vi "PrimaryProviderExample_CreateNewWizard_Invoke.vi"(10 "Cluster":T1, 11 "Wizard":T2) -> (3 "Canceled":bool)   [LabVIEW 2023]
uses:
  <resource>/Framework/Providers/API/ItemRef.ctl
  <resource>/Framework/Providers/API/mxLvNIIM.ctl
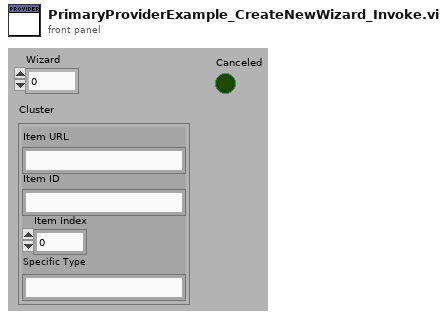
[diagram p1: front panel]
types:
  T1 = typedef "mxLvNIIM.ctl" = cluster{"Item URL":string, "Item ID":string, "Item Index":i32, "Specific Type":string}
  T2 = typedef "ItemRef.ctl" = u64
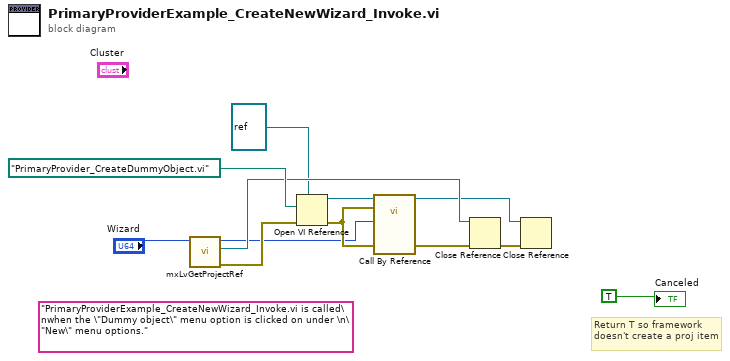
[diagram p0: block diagram]
diagram:
  (unwired) "PrimaryProviderExample_CreateNewWizard_Invoke.vi is called\nwhen the \"Dummy object\" menu option is clicked on under \n\"New\" menu options." ("message")
  # "Return T so framework\ndoesn't create a proj item"
  n1 = call <resource>:"mxLvGetProjectRef.vi"("Item"="Wizard") -> ("error out"=w10:errorcluster, "Project Refnum"=w8:refnum<vi>, "Item"=w3:T2)  [unwired: 8 in]
  n2 = Open VI Reference(type specifier VI Refnum (for type only)=refnum<vi> refnum, vi path=path "PrimaryProvider_CreateDummyObject.vi", error in (no error)=w10) -> (vi reference=w5:refnum<vi>, error out=w9:errorcluster)  [unwired: 3 in]
  n3 = call-by-ref "?"(reference=w5, error in=w9, 6:"error in (no error)"=w9, "Wizard"=w3) -> (reference out=w4:refnum<vi>, "error out"=w7:errorcluster)  [unwired: 6 in, 2 out]
  n4 = Close Reference(reference=w8, error in (no error)=w7) -> (error out=w2:errorcluster)
  n5 = Close Reference(reference=w4, error in (no error)=w2) -> ()  [unwired: 1 out]
  "Canceled" <- TRUE ("Canceled")
